vi "WaitForPopUpVIRef.vi"(0 "VI Reference In":refnum<vi>, 5 "Timeout(ms)":u32=10000, 11 "Error In":errorcluster) -> (4 "VI Reference Out":refnum<vi>, 15 "Error Out":errorcluster)   [LabVIEW 2019, in "Drona.lvlib"]
doc: "This VI waits until, the popup VI is the front most or timeout exceeds"
uses:
  Drona.lvlib
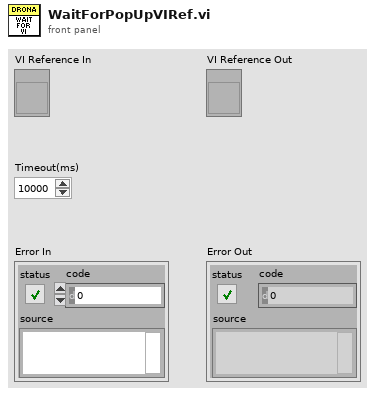
[diagram p1: front panel]
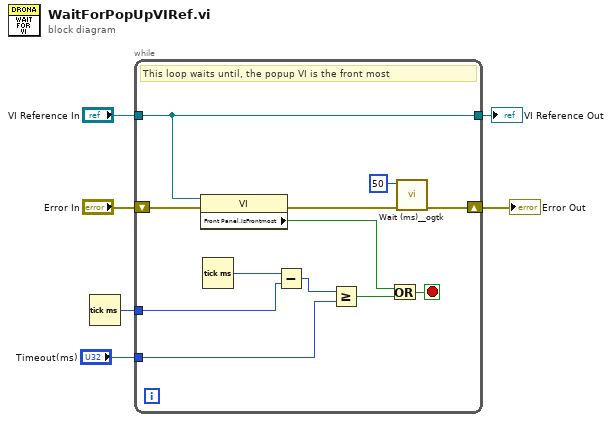
[diagram p0: block diagram]
diagram:
  n1 = Tick Count (ms)() -> (millisecond timer value=w4:u32)
  n2 = while {
    tunnel: "VI Reference In" -> [w8]
    tunnel: w4 -> [w18]
    tunnel: "Timeout(ms)" -> [w17]
    shift-right: [w12] -> w2
    shift-left: "Error In" -> [w10]
    tunnel: [w8] -> w1
    stop <- w13 stop-if-true
    # "This loop waits until, the popup VI is the front most"
    n3 = property class="VI"(reference=w8, error in=w10) -> (error out=w9:errorcluster, "Front Panel.IsFrontmost"=w7:bool)  [unwired: 1 out]
    n4 = Tick Count (ms)() -> (millisecond timer value=w16:u32)
    n5 = Subtract(x=w16, y=w18) -> (x-y=w15:u32)
    n6 = Greater Or Equal?(x=w15, y=w17) -> (x >= y?=w14:bool)
    n7 = Or(x=w7, y=w14) -> (x .or. y?=w13:bool)
    n8 = call <userlib>:"Wait (ms)__ogtk.vi"("error in (no error)"=w9, "milliseconds to wait"=u32 50) -> ("error out"=w12:errorcluster)  [unwired: 8 in, 1 out]
  }
  "Error Out" <- w2
  "VI Reference Out" <- w1
